vi "NR recall Param.vi"(8 "error in (no error)":errorcluster caption="에러 입력(에러 없음)", 10 "Recall Name":string, 11 "Instrument Manager 입력":refnum<class "Instrument Manager.lvclass">) -> (0 "error out":errorcluster caption="에러 출력", 3 "Instrument Manager 출력":refnum<class "Instrument Manager.lvclass">)   [LabVIEW 2023, in "Instrument Manager.lvclass"]
uses:
  Instrument Manager.lvclass
  Instrument Manager.lvclass/Instrument Manager.ctl
  Module/ANRITSU Call Box/Interface Class/Anritsu Call Box.lvclass
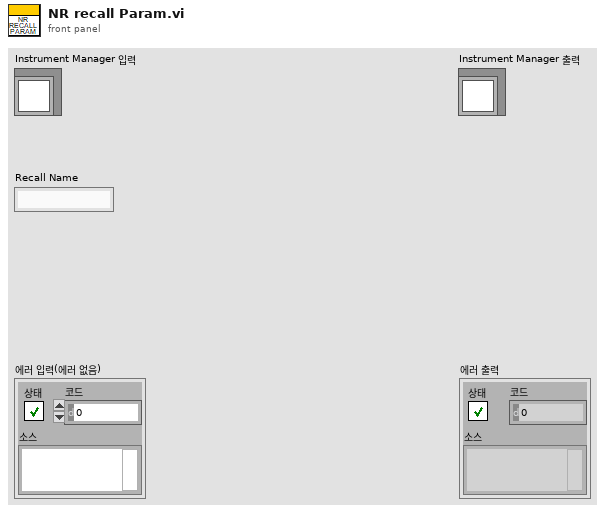
[diagram p1: front panel]
types:
  T1 = cluster{"Anritsu Call Box":refnum<class "Anritsu Call Box.lvclass">, "Spectrum Analyzer":refnum<class "Interface_Spectrum.lvclass">, "RF Switch Box":refnum<class "RF Filter Box.lvclass">, "Turn Table":refnum<class "Interface - Turn Table.lvclass">, "Mast":refnum<class "Interface - Mast.lvclass">, "3D Controller":refnum<class "Interface_3D Controller.lvclass">}
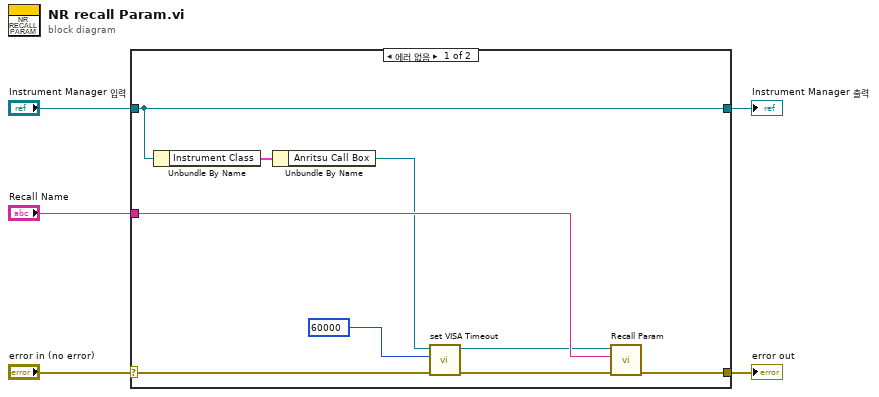
[diagram p0: block diagram]
diagram:
  n1 = case shown="에러 없음" "error in (no error)" {
    selector: "error in (no error)" -> [w10 w16]
    tunnel: [w14 w16] -> w4
    tunnel: [w13 w15] -> w2
    tunnel: "Instrument Manager 입력" -> [w13 w15]
    tunnel: "Recall Name" -> [w11 _]
    frame No Error {
      n2 = Unbundle By Name(w13) -> ("Instrument Class"=w12:T1)
      n3 = Unbundle By Name(w12) -> ("Anritsu Call Box"=w8:refnum<class "Anritsu Call Box.lvclass">)
      n4 = call-dynamic "set VISA Timeout.vi"("error in (no error)"=w10, "Timeout Value"=u32 60000, "Anritsu Call Box 입력"=w8) -> ("error out"=w9:errorcluster, "Anritsu Call Box 출력"=w7:refnum<class "Anritsu Call Box.lvclass">)  [unwired: 7 in]
      n5 = call-dynamic "Recall Param.vi"("error in (no error)"=w9, "Recall Name"=w11, "Anritsu Call Box 입력"=w7) -> ("error out"=w14:errorcluster)  [unwired: 7 in, 1 out]
    }
    frame Error {
    }
  }
  "error out" <- w4
  "Instrument Manager 출력" <- w2
